vi "Summary.vi"(8 "error in":errorcluster, 10 "depth":i32, 11 "node self ref":T1) -> (0 "error out":errorcluster, 2 "summary":T2[](array[typedef]))   [LabVIEW 2014, in "NISE_CEF_TreeControl.lvlib"]
doc: "Gets the summary of a node and all the subnodes. This description can be used to update the tree control"
uses:
  NISE_CEF_TreeControl.lvlib
  Node/Summary.ctl
  Node/NodeRef.ctl
  Node/NISE_CEF_Node.lvclass
  Node/NISE_CEF_Node.lvclass/NISE_CEF_Node.ctl
  Node/ReadParent.vi
  Node/ReadChildren.vi
  Node/ReadNodeClass.vi
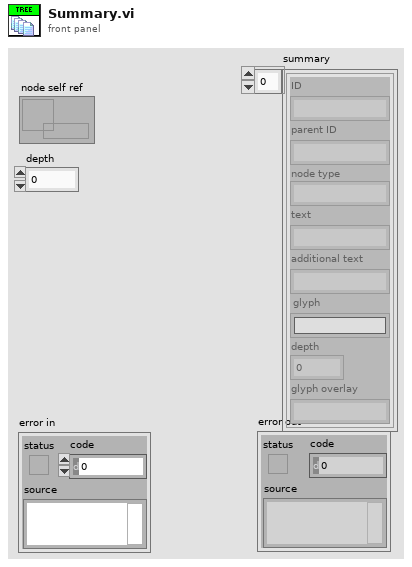
[diagram p1: front panel]
types:
  T1 = typedef "NISE_CEF_Node.lvclass/NodeRef.ctl" = refnum<data-value>
  T2 = typedef "NISE_CEF_Node.lvclass/Summary.ctl" = cluster{"ID":string, "parent ID":string, "node type":string, "text":string, "additional text":string, "glyph":string, "depth":i32, "glyph overlay":string}
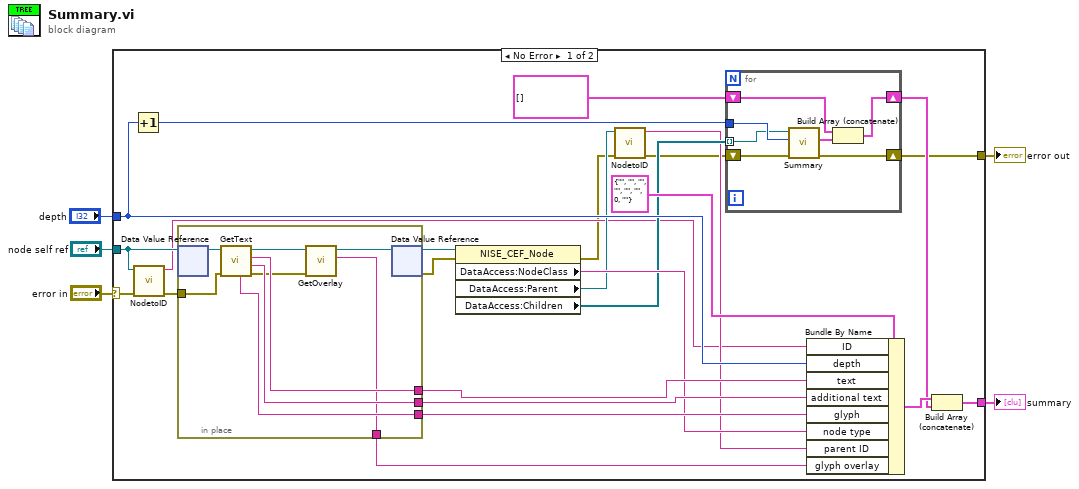
[diagram p0: block diagram]
diagram:
  n1 = case shown="No Error" "error in" {
    selector: "error in" -> [w13 w46]
    tunnel: [w7 w46] -> w4
    tunnel: "node self ref" -> [w15 _]
    tunnel: "depth" -> [w29 _]
    tunnel: [w28 _] -> w1
    frame No Error {
      n2 = Increment(x=w29) -> (x+1=w22:i32)
      n3 = call "NodetoID.vi"("error in"=w13, "node ref"=w15) -> ("error out"=w12:errorcluster, "ID"=w14:string)  [unwired: 8 in]
      n4 = in-place {
        in-place-border: [w38] -> w26
        in-place-border: [w37] -> w25
        in-place-border: [w36] -> w24
        in-place-border: w12 -> [w35]
        in-place-border: [w30] -> w6
        n5 = in-place-dvr #1(w15) -> (w34:refnum<class "NISE_CEF_Node.lvclass">)  [unwired: 1 out]
        n6 = call-dynamic "GetText.vi"("error in"=w35, "node in"=w34) -> ("error out"=w31:errorcluster, "additional text"=w38:string, "text"=w37:string, "node out"=w33:refnum<class "NISE_CEF_Node.lvclass">, "glyph"=w36:string)  [unwired: 5 in]
        n7 = call-dynamic "GetOverlay.vi"("error in"=w31, "NISE_CEF_Node in"=w33) -> ("overlay"=w30:string, "NISE_CEF_Node out"=w32:refnum<class "NISE_CEF_Node.lvclass">)  [unwired: 7 in, 1 out]
        n8 = in-place-dvr #1(w32) -> (w11:T1, w10:errorcluster)
      }
      n9 = property class="NISE_CEF_Node"(reference=w11, error in=w10) -> (error out=w9:errorcluster, "DataAccess:NodeClass"=w23:string, "DataAccess:Parent"=w17:T1, "DataAccess:Children"=w18:T1[])  [unwired: 1 out]
      n10 = call "NodetoID.vi"("error in"=w9, "node ref"=w17) -> ("error out"=w8:errorcluster, "ID"=w16:string)  [unwired: 8 in]
      n11 = for {
        tunnel: w18 -> [w41] mode=indexing
        tunnel: w22 -> [w45]
        shift-right: [w43] -> w19
        shift-left: T2[] [] ("childrensummary") -> [w44]
        shift-right: [w39] -> w7
        shift-left: w8 -> [w40]
        n12 = call "Summary.vi"("error in"=w40, "depth"=w45, "node self ref"=w41) -> ("error out"=w39:errorcluster, "summary"=w42:T2[])  [unwired: 7 in]
        n13 = Build Array (concatenate)(w44, w42) -> (w43:T2[])
      }
      n14 = Bundle By Name(cluster=T2 {"ID"="", "parent ID"="", "node type"="", "text"="", "additional text"="", "glyph"="", "depth"=0, "glyph overlay"=""} ("nodeSummary"), "ID"=w14, "depth"=w29, "text"=w25, "additional text"=w26, "glyph"=w24, "node type"=w23, "parent ID"=w16, "glyph overlay"=w6) -> (w20:T2)
      n15 = Build Array (concatenate)(w20, w19) -> (w28:T2[])
    }
    frame Error {
    }
  }
  "error out" <- w4
  "summary" <- w1
